vi "test category list.vi"() -> ()   [LabVIEW 2014]
doc: "::: VI Helpeks :::\nCopyright (c) 2000-2026 Konstantin Shifershteyn. All rights reserved."
panel:
  in  "Category List 2":i32(listbox)
  in  "Category List":i32(listbox)
  # "VI Helpeks\nCopyright (c) 2012-2026 Konstantin Shifershteyn"
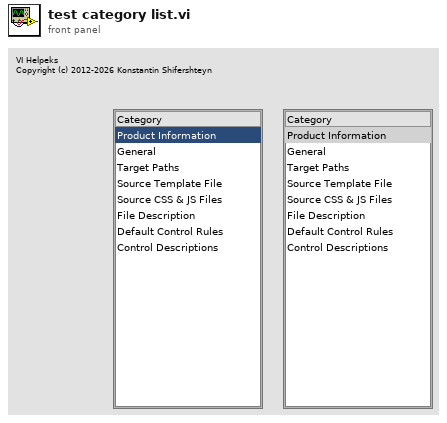
[diagram p1: front panel]
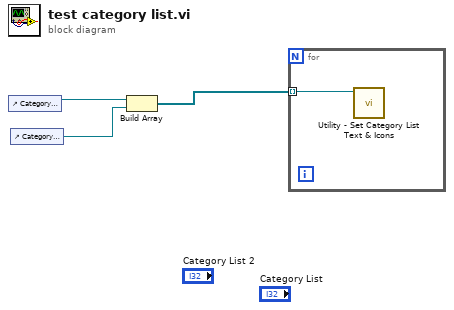
[diagram p0: block diagram]
diagram:
  n1 = control-ref of="Category List"() -> (w3:refnum<vi>)
  n2 = control-ref of="Category List 2"() -> (w2:refnum<vi>)
  n3 = Build Array(w3, w2) -> (w1:refnum<vi>[])
  n4 = for {
    tunnel: w1 -> [w4] mode=indexing
    n5 = call "Utility - Set Category List Text & Icons.vi"("LstBox Refnum"=w4) -> ()  [unwired: 10 in, 1 out]
  }
